vi "Convert Cluster Array to Waveform Array.vi"(11 "input data":cluster{"t0":dbl, "dt":dbl, "Y":dbl[]}[](array[cluster])) -> (3 "waveforms out":waveform(dbl)[](array[waveform]))   [LabVIEW 2026]
doc: "Converts a 1D array of clusters {t0, dt, Y} into a 1D array of waveform DBL."
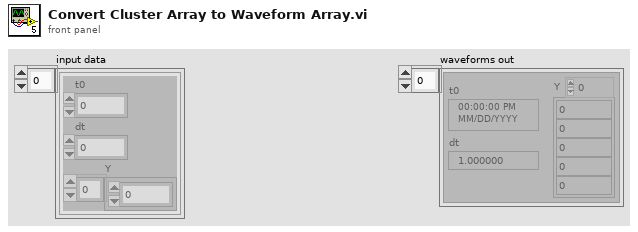
[diagram p1: front panel]
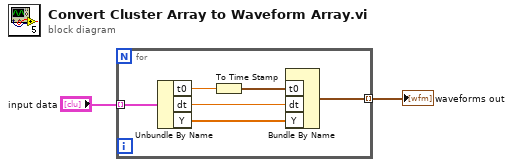
[diagram p0: block diagram]
diagram:
  n1 = for {
    tunnel: "input data" -> [w8] mode=indexing
    tunnel: [w3] -> w1 mode=indexing
    n2 = Unbundle By Name(w8) -> ("t0"=w7:dbl, "dt"=w5:dbl, "Y"=w4:dbl[])
    n3 = To Time Stamp(1:w7) -> (0:w6:timestamp)
    n4 = Bundle By Name("t0"=w6, "dt"=w5, "Y"=w4) -> (w3:waveform(dbl))  [unwired: 1 in]
  }
  "waveforms out" <- w1
